vi "JsonRpcRequestStringToCluster.vi"(8 "error in (no error)":errorcluster, 10 "JsonRpcHttpRequestBodyString":string) -> (0 "error out":errorcluster, 2 "JsonRPCHttpRequestBody":T1)   [LabVIEW 2017]
uses:
  <vilib>/LVH/i3 JSON/JSON Parsing/Get Object Parameter Files/Get Object Parameter - String.vi
  <vilib>/LVH/i3 JSON/JSON Parsing/Get Object Parameter Files/Get Object Parameter - JSON Tree.vi
  <vilib>/LVH/i3 JSON/i3-json.lvlib
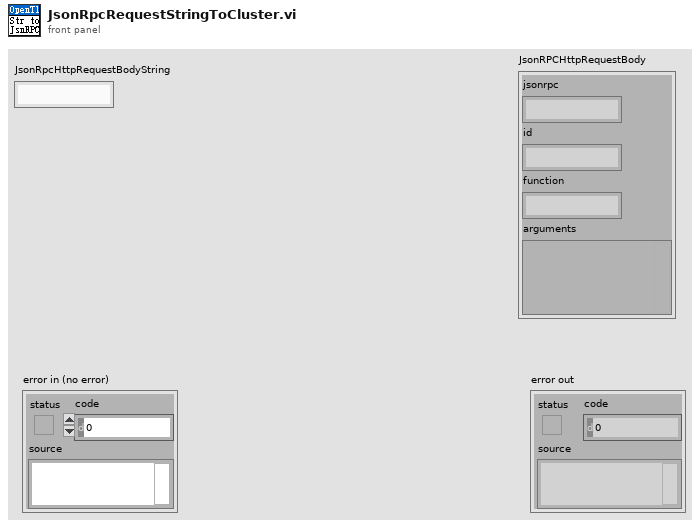
[diagram p1: front panel]
types:
  T1 = cluster{"jsonrpc":string, "id":string, "function":string, "arguments":variant}
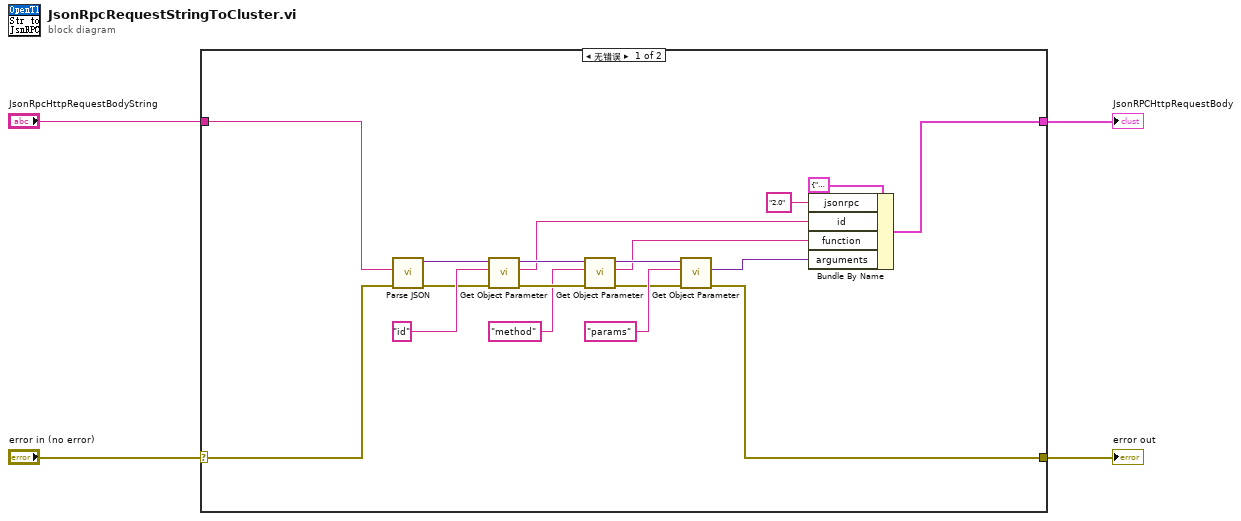
[diagram p0: block diagram]
diagram:
  n1 = case shown="无错误" "error in (no error)" {
    selector: "error in (no error)" -> [w12 w23]
    tunnel: [w5 w23] -> w3
    tunnel: "JsonRpcHttpRequestBodyString" -> [w13 _]
    tunnel: [w6 _] -> w1
    frame No Error {
      n2 = call <vilib>:"Parse JSON.vi"("error in (no error)"=w12, "JSON String"=w13) -> ("error out"=w20:errorcluster, "JSON Tree"=w22:variant)  [unwired: 6 in, 2 out]
      n3 = call-poly <vilib>:"Get Object Parameter.vi"("error in (no error)"=w20, "Parameter Name"="id", "JSON Tree In (JSON Object)"=w22) -> ("error out"=w18:errorcluster, "String Value"=w9:string, "JSON Tree Out Passthrough"=w19:variant)  [unwired: 5 in, 1 out]
      n4 = call-poly <vilib>:"Get Object Parameter.vi"("error in (no error)"=w18, "Parameter Name"="method", "JSON Tree In (JSON Object)"=w19) -> ("error out"=w14:errorcluster, "String Value"=w8:string, "JSON Tree Out Passthrough"=w16:variant)  [unwired: 5 in, 1 out]
      n5 = call-poly <vilib>:"Get Object Parameter.vi"("error in (no error)"=w14, "Parameter Name"="params", "JSON Tree In (JSON Object)"=w16) -> ("error out"=w5:errorcluster, "JSON Value (JSON Tree)"=w7:variant)  [unwired: 5 in, 2 out]
      n6 = Bundle By Name(cluster=T1 {"jsonrpc"="", "id"="", "function"="", "arguments"=variant} ("JsonRPCHttpRequestBody"), "jsonrpc"="2.0", "id"=w9, "function"=w8, "arguments"=w7) -> (w6:T1)
    }
    frame Error {
    }
  }
  "error out" <- w3
  "JsonRPCHttpRequestBody" <- w1
